vi "GV-SetGraphData.vi"(8 "error in (no error)":errorcluster, 9 "GviewerUpdate":T1, 11 "Gviewer in":refnum<class "Gviewer.lvclass">) -> (0 "error out":errorcluster, 3 "Gviewer out":refnum<class "Gviewer.lvclass">)   [LabVIEW 2020, in "Sgraph_lib_V1.lvlib" / "Gviewer.lvclass"]
doc: "Andre Koelewijn, 17 jan 2021\n\nWrite Graph data"
uses:
  Gviewer.lvclass
  FAMM/controls/FAMM_reply_datagram.ctl
  controls/Typedef_Live.ctl
  FAMM/controls/FAMM_reply_WAQdata.ctl
  FAMM/controls/FAMM_reply_EAQdata.ctl
  FAMM/controls/FAMM_reply_PAQdata.ctl
  Gviewer.lvclass/Gviewer.ctl
  FAMM/FAMM.lvclass
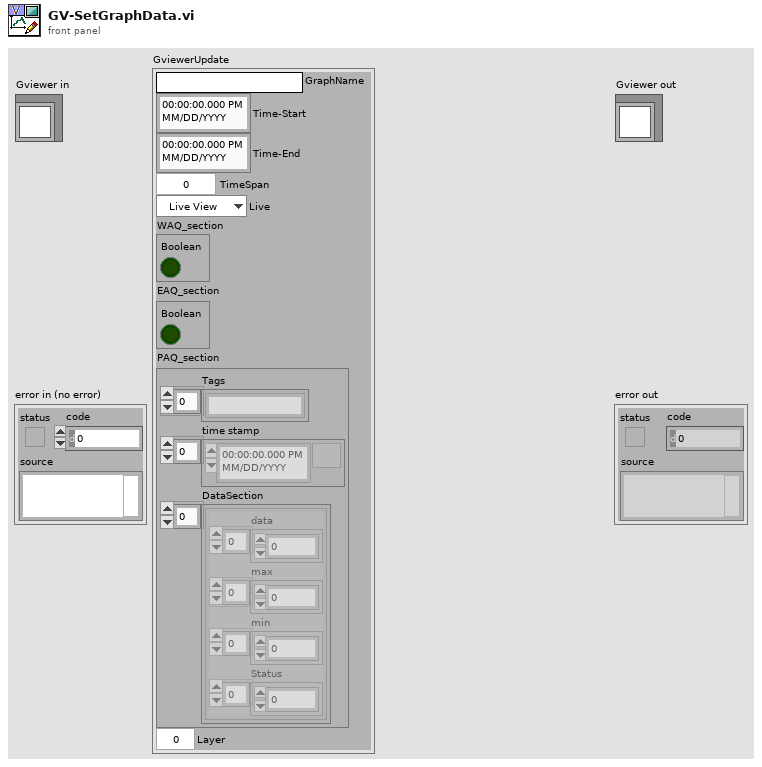
[diagram p1: front panel]
types:
  T1 = typedef "Sgraph_lib_V1.lvlib/FAMM.lvclass/FAMM_reply_datagram.ctl" = cluster{"GraphName":string, "Time-Start":timestamp, "Time-End":timestamp, "TimeSpan":dbl, "Live":T2, "WAQ_section":T3, "EAQ_section":T4, "PAQ_section":T5, "Layer":i32}
  T2 = typedef "Sgraph_lib_V1.lvlib/Gviewer.lvclass/Typedef_Live.ctl" = enum16{"Live View", "Freeze"}
  T3 = typedef "Sgraph_lib_V1.lvlib/FAMM.lvclass/FAMM_reply_WAQdata.ctl" = cluster{"Boolean":bool}
  T4 = typedef "Sgraph_lib_V1.lvlib/FAMM.lvclass/FAMM_reply_EAQdata.ctl" = cluster{"Boolean":bool}
  T5 = typedef "Sgraph_lib_V1.lvlib/FAMM.lvclass/FAMM_reply_PAQdata.ctl" = cluster{"Tags":string[], "time stamp":timestamp[], "DataSection":cluster{"data":dbl[], "max":dbl[], "min":dbl[], "Status":u32[]}[]}
  T6 = typedef "Sgraph_lib_V1.lvlib/Gviewer.lvclass/Typedef_SelProperties.ctl" = cluster{"Color":u32, "LineType":T7, "max":dbl, "min":dbl}
  T7 = typedef "Sgraph_lib_V1.lvlib/Gviewer.lvclass/Typedef_LineType.ctl" = enum16{"num_bare", "num_MinMax_Area", "num_MinMax_Lines", "num_MinMax_Forfor", "num_Max_Area", "num_Max_Line", "num_Max_Forfor", "num_Min_Area", "num_Min_Line", "num_Min_Fosfor", "Boolean_Line_01", "Boolean_Area_01", "Boolean_Fosfor_01", "Boolean_Line_TF", "Boolean_Area_TF", "Boolean_Fosfor_TF", "Boolean_OnOff_Line", "Boolean_OnOff_Area", "Boolean_OnOff_Fosfor", "Boolean_spare", "StringEvent_Line", "StringEvent_TimeLine"}
  T8 = cluster{"data":dbl[], "max":dbl[], "min":dbl[], "Status":u32[]}[]
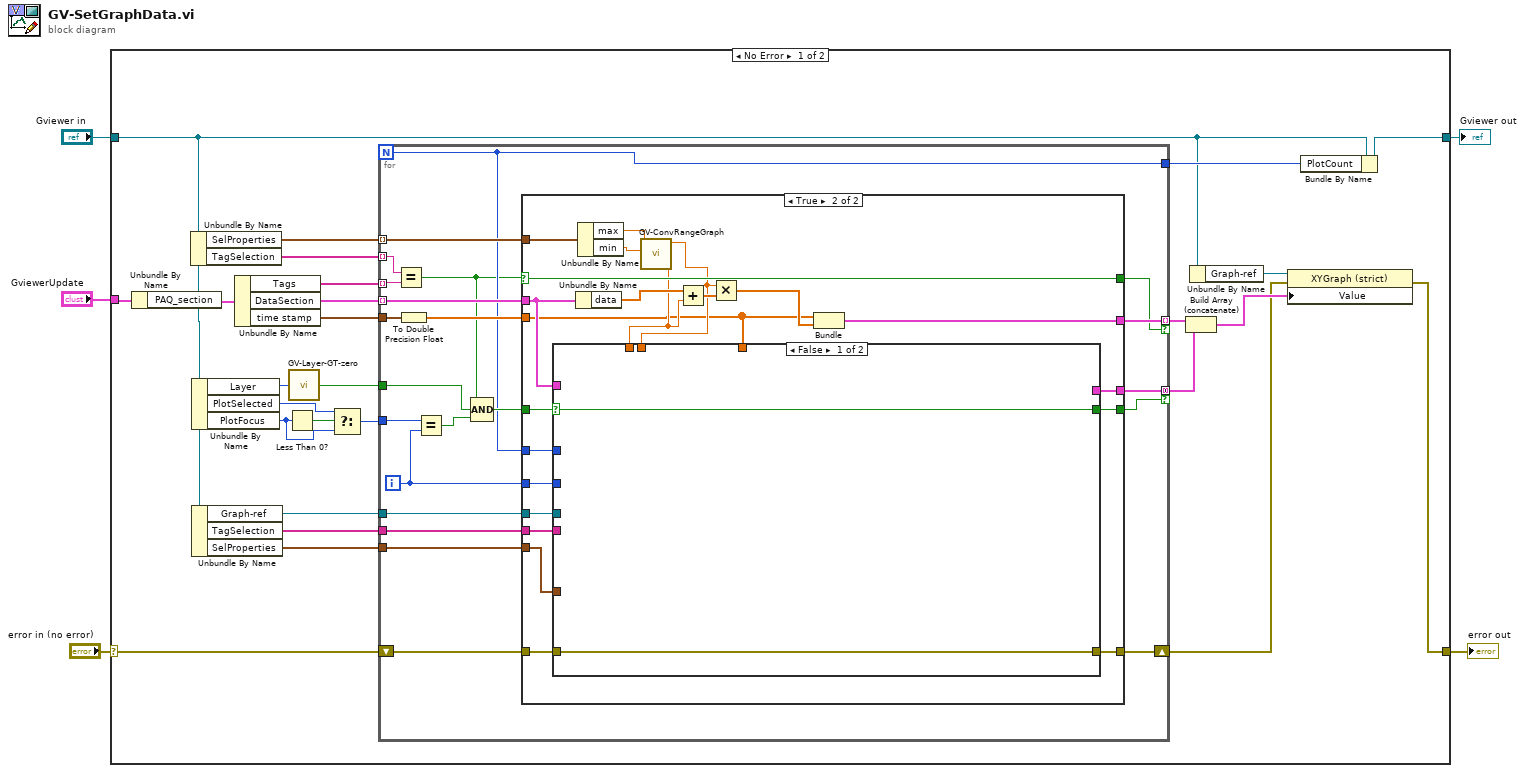
[diagram p0: block diagram]
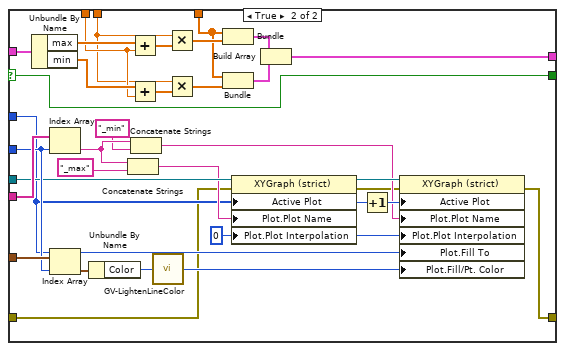
[diagram p3: hidden frame]
diagram:
  n1 = case shown="No Error" "error in (no error)" {
    selector: "error in (no error)" -> [w12 w114]
    tunnel: [w24 w114] -> w4
    tunnel: [w21 w113] -> w2
    tunnel: "Gviewer in" -> [w16 w113]
    tunnel: "GviewerUpdate" -> [w22 _]
    frame No Error {
      n2 = Unbundle By Name(w22) -> ("PAQ_section"=w30:T5)
      n3 = Unbundle By Name(w16) -> ("SelProperties"=w23:T6[], "TagSelection"=w26:string[])
      n4 = Unbundle By Name(w16) -> ("Layer"=w7:i32, "PlotSelected"=w9:i32, "PlotFocus"=w10:i32)
      n5 = Unbundle By Name(w16) -> ("Graph-ref"=w13:refnum<vi>, "TagSelection"=w15:string[], "SelProperties"=w14:T6[])
      n6 = Unbundle By Name(w30) -> ("Tags"=w29:string[], "DataSection"=w28:T8, "time stamp"=w27:timestamp[])
      n7 = Less Than 0?(x=w10) -> (x < 0?=w11:bool)
      n8 = call "GV-Layer-GT-zero.vi"("Layer"=w7) -> (">0 ?"=w6:bool)  [unwired: 8 in]
      n9 = Select(t=w9, s=w11, f=w10) -> (s? t:f=w8:i32)
      n10 = for {
        N -> [w38]
        tunnel: w29 -> [w52] mode=indexing
        tunnel: w28 -> [w50] mode=indexing
        tunnel: w27 -> [w49]
        tunnel: w26 -> [w51] mode=indexing
        tunnel: [w48] -> w18 mode=indexing if=w45
        tunnel: w23 -> [w46] mode=indexing
        tunnel: [w38] -> w20
        tunnel: [w44] -> w17 mode=concatenating if=w42
        tunnel: w15 -> [w41]
        tunnel: w14 -> [w40]
        tunnel: w13 -> [w39]
        shift-right: [w36] -> _
        shift-left: w12 -> [w37]
        tunnel: w6 -> [w34]
        tunnel: w8 -> [w31]
        i -> [w33]
        n11 = Equal?(x=w51, y=w52) -> (x = y?=w35:bool)
        n12 = To Double Precision Float(number=w49) -> (double precision float=w47:dbl[])
        n13 = Equal?(x=w31, y=w33) -> (x = y?=w32:bool)
        n14 = Compound Arithmetic op=AND(w35, w34, w32) -> (w43:bool)
        n15 = case shown="True" w35 {
          selector: w35 -> [w55 w76]
          tunnel: w50 -> [_ w69]
          tunnel: w47 -> [_ w66]
          tunnel: [_ w77] -> w48
          tunnel: [w55 w76] -> w45
          tunnel: w46 -> [_ w75]
          tunnel: [_ w65] -> w44
          tunnel: w43 -> [w54 w64]
          tunnel: [w54 w63] -> w42
          tunnel: w41 -> [_ w62]
          tunnel: w40 -> [_ w61]
          tunnel: w33 -> [_ w60]
          tunnel: w39 -> [_ w59]
          tunnel: w38 -> [_ w58]
          tunnel: w37 -> [w53 w57]
          tunnel: [w53 w56] -> w36
          frame False {
          }
          frame True {
            n16 = Unbundle By Name(w69) -> ("data"=w72:dbl[])
            n17 = Unbundle By Name(w75) -> ("max"=w74:dbl, "min"=w73:dbl)
            n18 = call "GV-ConvRangeGraph.vi"("RangeL"=w73, "RangeH"=w74) -> ("Offset"=w68:dbl, "Gain"=w67:dbl)  [unwired: 8 in]
            n19 = case shown="False" w64 {
              selector: w64 -> [w79 w99]
              tunnel: w69 -> [_ w106]
              tunnel: w68 -> [_ w105]
              tunnel: w67 -> [_ w104]
              tunnel: w66 -> [_ w103]
              tunnel: [_ w100] -> w65
              tunnel: [w79 w99] -> w63
              tunnel: w62 -> [_ w98]
              tunnel: w61 -> [_ w97]
              tunnel: w60 -> [_ w96]
              tunnel: w59 -> [_ w93]
              tunnel: w58 -> [_ w84]
              tunnel: w57 -> [w78 w82]
              tunnel: [w78 w80] -> w56
              frame False {
              }
              frame True {
                w85 = u8 0 ("Plot.Plot Interpolation")
                n20 = Unbundle By Name(w106) -> ("max"=w112:dbl[], "min"=w111:dbl[])
                n21 = Index Array(array=w98, index=w96) -> (element=w90:string)
                n22 = Index Array(array=w97, index=w96) -> (element=w95:T6)
                n23 = Unbundle By Name(w95) -> ("Color"=w94:u32)
                n24 = Concatenate Strings(w90, "_max") -> (w86:string)
                n25 = Add(x=w112, y=w105) -> (x+y=w110:dbl[])
                n26 = Add(x=w111, y=w105) -> (x+y=w109:dbl[])
                n27 = Concatenate Strings(w90, "_min") -> (w87:string)
                n28 = call "GV-LightenLineColor.vi"("Line color"=w94) -> ("Light color"=w83:u32)  [unwired: 6 in]
                n29 = Multiply(x=w104, y=w110) -> (x*y=w108:dbl[])
                n30 = Multiply(x=w104, y=w109) -> (x*y=w107:dbl[])
                n31 = Bundle(w103, w108) -> (w102:cluster{dbl[], dbl[]})  [unwired: 1 in]
                n32 = Bundle(w103, w107) -> (w101:cluster{dbl[], dbl[]})  [unwired: 1 in]
                n33 = property class="XYGraph (strict)"(reference=w93, error in=w82, "Active Plot"=w84, "Plot.Plot Name"=w86, "Plot.Plot Interpolation"=w85) -> (reference out=w92:refnum<vi>, error out=w81:errorcluster)
                n34 = Build Array(w102, w101) -> (w100:cluster{dbl[], dbl[]}[])
                n35 = Increment(x=w84) -> (x+1=w91:i32)
                n36 = property class="XYGraph (strict)"(reference=w92, error in=w81, "Active Plot"=w91, "Plot.Plot Name"=w87, "Plot.Plot Interpolation"=w85, "Plot.Fill To"=w84, "Plot.Fill/Pt. Color"=w83) -> (error out=w80:errorcluster)  [unwired: 1 out]
              }
            }
            n37 = Add(x=w72, y=w68) -> (x+y=w71:dbl[])
            n38 = Multiply(x=w67, y=w71) -> (x*y=w70:dbl[])
            n39 = Bundle(w66, w70) -> (w77:cluster{dbl[], dbl[]})  [unwired: 1 in]
          }
        }
      }
      n40 = Build Array (concatenate)(w18, w17) -> (w19:cluster{dbl[], dbl[]}[])
      n41 = Unbundle By Name(w16) -> ("Graph-ref"=w25:refnum<vi>)
      n42 = property class="XYGraph (strict)"(reference=w25, error in=w12, "Value"=w19) -> (error out=w24:errorcluster)  [unwired: 1 out]
      n43 = Bundle By Name(cluster=w16, "PlotCount"=w20) -> (w21:refnum<class "Gviewer.lvclass">)
    }
    frame Error {
    }
  }
  "error out" <- w4
  "Gviewer out" <- w2
